vi "test_DMA Channels Input.vi"(8 "error in (no error)":errorcluster, 11 "TestCase in":refnum<class "FPGA Addon DMA Channel Unit Tests.lvclass">) -> (0 "error out":errorcluster, 3 "TestCase out":refnum<class "FPGA Addon DMA Channel Unit Tests.lvclass">)   [LabVIEW 2020, in "FPGA Addon DMA Channel Unit Tests.lvclass"]
uses:
  FPGA Addon DMA Channel Unit Tests.lvclass
  Addon/Addon Shared/Types/DMA Settings.ctl
  Addon/Addon Shared/Types/Delacing Scheme.ctl
  Addon/Addon Shared/Types/DMA Acquisition Mode.ctl
  FPGA Addon DMA Channel Unit Tests.lvclass/FPGA Addon DMA Channel Unit Tests.ctl
  Addon/Addon Shared/SubVIs/Constants.vi
  <vilib>/NI/NI VeriStand Advanced SysDef API/_SubVIs/SysDef.Search.GUID.vi
  <vilib>/NI/NI VeriStand Advanced SysDef API/_SubVIs/SysDef.Search.GUIDs.vi
  <vilib>/addons/_JKI Toolkits/VI Tester/TestCase.llb/TestCase.lvclass
  Addon/Addon System Explorer/FPGA Addon System Explorer.lvlib
  Addon/Addon Shared/FPGA Addon Shared.lvlib
  <vilib>/NI/NI VeriStand Advanced SysDef API/SysDef API/Advanced System Definition.lvlib
  C:/Program Files (x86)/National Instruments/LabVIEW 2020/vi.lib/addons/_JKI Toolkits/VI Tester/TestCase.llb/TestCase.lvclass
panel:
  out "error out 2":errorcluster
  out "Array":string[](array[string])
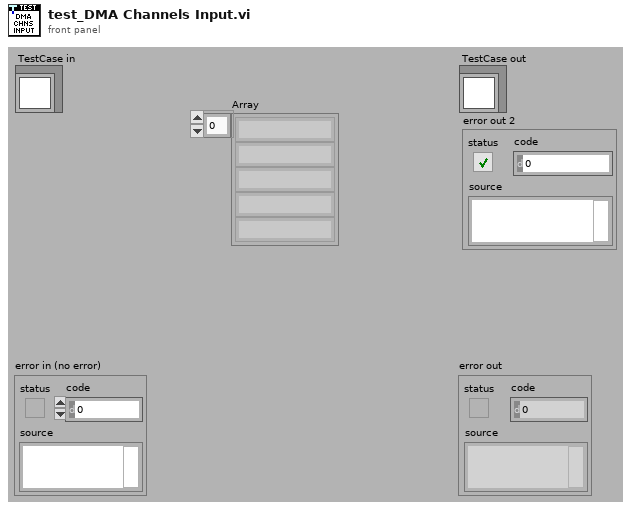
[diagram p1: front panel]
types:
  T1 = typedef "FPGA Addon Shared.lvlib/DMA Settings.ctl" = cluster{"Number of Channels":u8, "Delacing Scheme":T2, "Update Rate":u32, "dt":dbl, "Mode":T3, "Number of Samples":u32, "DMA Host Buffer":u32}
  T2 = typedef "FPGA Addon Shared.lvlib/Delacing Scheme.ctl" = enum8{"Interleaved", "Bitpacked"}
  T3 = typedef "FPGA Addon Shared.lvlib/DMA Acquisition Mode.ctl" = enum8{"Continuous", "Triggered Finite"}
  T4 = typedef "Advanced System Definition.lvlib/TreeItem.Info.ctl" = cluster{"Name":string, "Description":string, "GUID":string, "Is Channel":bool, "Channel":T5, "Is Waveform":bool, "Waveform":T7}
  T5 = typedef "Custom Device API.lvlib/Custom Device Channel.ctl" = cluster{"Type":T6, "Units":string, "Default Value":dbl, "Faultable":bool, "Scalable":bool}
  T6 = typedef "Custom Device API.lvlib/Custom Device Channel Type.ctl" = enum16{"Input", "Output"}
  T7 = typedef "Custom Device API.lvlib/Custom Device Waveform.ctl" = cluster{"Data Type":T8, "Units":string}
  T8 = typedef "Custom Device API.lvlib/Custom Device Waveform DataType.ctl" = enum16{"Double", "Complex Double"}
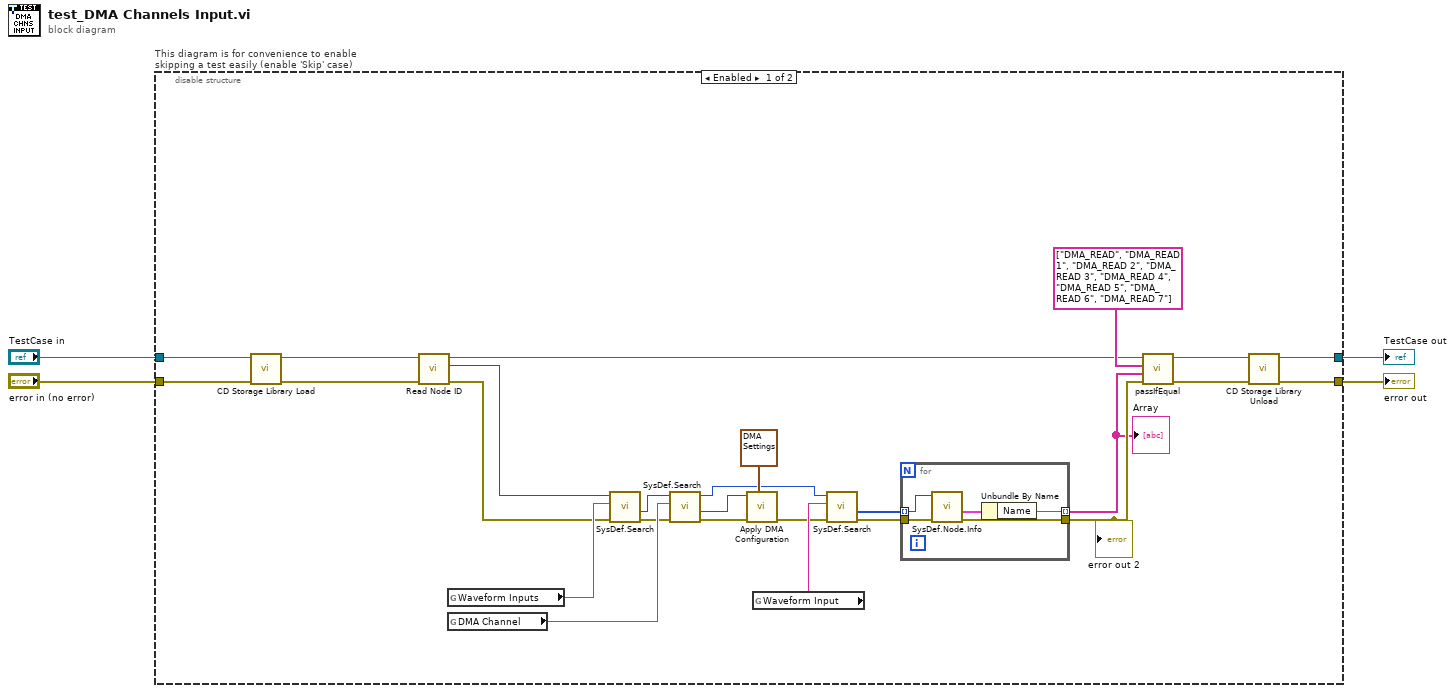
[diagram p0: block diagram]
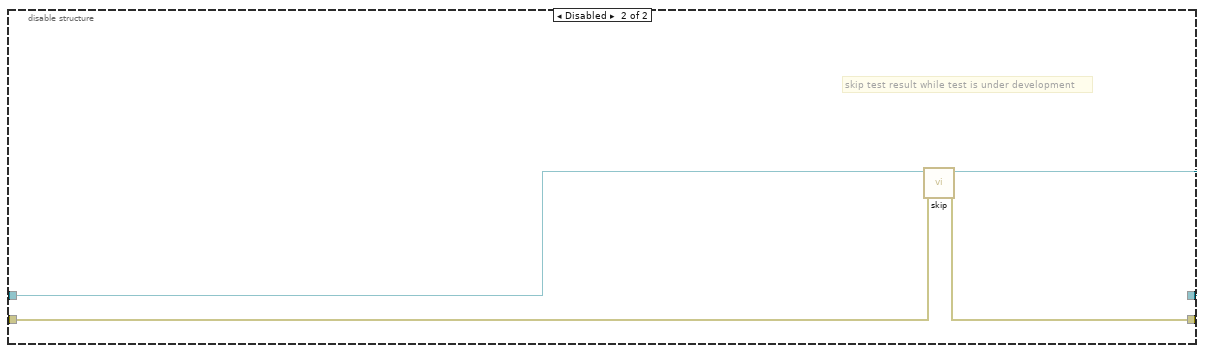
[diagram p2: hidden frame]
diagram:
  n1 = disable-structure "This diagram is for convenience to enable skipping a test easily (enable 'Skip' case)" shown="Enabled" {
    disable-tunnel: "TestCase in" -> [w13 w39]
    disable-tunnel: [w7 w37] -> w1
    disable-tunnel: [w8 w38] -> w3
    disable-tunnel: "error in (no error)" -> [w14 w36]
    frame Enabled {
      n2 = call "CD Storage Library Load.vi"("error in (no error)"=w14, "DMA Channel Testing in"=w13) -> ("error out"=w11:errorcluster, "DMA Channel Testing out"=w12:refnum<class "FPGA Addon DMA Channel Unit Tests.lvclass">)  [unwired: 8 in]
      n3 = call "Read Node ID.vi"("error in (no error)"=w11, "DMA Channel Testing in"=w12) -> ("error out"=w17:errorcluster, "Node ID"=w16:u64, "DMA Channel Testing out"=w15:refnum<class "FPGA Addon DMA Channel Unit Tests.lvclass">)  [unwired: 7 in]
      n4 = global read "Constants.vi" "Waveform Inputs"() -> (w29:string)
      n5 = global read "Constants.vi" "DMA Channel"() -> (w28:string)
      n6 = call-poly <vilib>:"SysDef.Search.vi"("error in (no error)"=w17, "GUID"=w29, "nodeID"=w16) -> ("error out"=w26:errorcluster, "Value out"=w27:u64)  [unwired: 5 in, 2 out]
      n7 = call-poly <vilib>:"SysDef.Search.vi"("error in (no error)"=w26, "GUID"=w28, "nodeID"=w27) -> ("error out"=w6:errorcluster, "Value out"=w25:u64, "nodeID out"=w23:u64)  [unwired: 5 in, 1 out]
      n8 = call "Apply DMA Configuration.vi"("DMA Settings"=T1 {"Number of Channels"=8, "Delacing Scheme"=enum."Interleaved", "Update Rate"=0, "dt"=0.0, "Mode"=enum."Continuous", "Number of Samples"=0, "DMA Host Buffer"=0}, "error in (no error)"=w6, "Item Ref in"=w25) -> ("error out"=w5:errorcluster)  [unwired: 8 in]
      n9 = global read "Constants.vi" "Waveform Input"() -> (w24:string)
      n10 = call-poly <vilib>:"SysDef.Search.vi"("error in (no error)"=w5, "GUID"=w24, "nodeID"=w23) -> ("error out"=w21:errorcluster, "Values Out"=w22:u64[])  [unwired: 5 in, 2 out]
      n11 = for {
        tunnel: w22 -> [w35] mode=indexing
        tunnel: w21 -> [w34]
        tunnel: [w33] -> w20
        tunnel: [w31] -> w19 mode=indexing
        n12 = call <vilib>:"SysDef.Node.Info.vi"("error in (no error)"=w34, "nodeID"=w35) -> ("error out"=w33:errorcluster, "Item Info"=w32:T4)  [unwired: 6 in, 2 out]
        n13 = Unbundle By Name(w32) -> ("Name"=w31:string)
      }
      "Array" <- w19
      "error out 2" <- w20
      n14 = call-dynamic "passIfEqual.vi"("error in (no error)"=w20, "y"=w19, "x"=string[] ["DMA_READ", "DMA_READ 1", "DMA_READ 2", "DMA_READ 3", "DMA_READ 4", "DMA_READ 5", "DMA_READ 6", "DMA_READ 7"] ("Array"), "TestCase in"=w15) -> ("error out"=w10:errorcluster, "TestCase out"=w9:refnum<class "FPGA Addon DMA Channel Unit Tests.lvclass">)  [unwired: 6 in]
      n15 = call "CD Storage Library Unload.vi"("error in (no error)"=w10, "DMA Channel Testing in"=w9) -> ("error out"=w8:errorcluster, "DMA Channel Testing out"=w7:refnum<class "FPGA Addon DMA Channel Unit Tests.lvclass">)  [unwired: 8 in]
    }
    frame Disabled {
      # "skip test result while test is under development"
      n16 = call <vilib>:"skip.vi"("error in (no error)"=w36, "TestCase in"=w39) -> ("error out"=w38:errorcluster, "TestCase out"=w37:refnum<class "FPGA Addon DMA Channel Unit Tests.lvclass">)  [unwired: 8 in]
    }
  }
  "error out" <- w3
  "TestCase out" <- w1
